vi "I2C Message Buffer - Check.vi"(8 "error in (no error)":errorcluster) -> (0 "error out":errorcluster, 2 "Messages":i32, 3 "Transactions":i32)   [LabVIEW 2025, in "I2C Bus Monitor.lvclass"]
uses:
  I2C Bus Monitor.lvclass
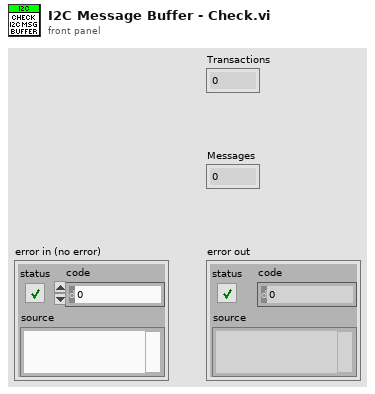
[diagram p1: front panel]
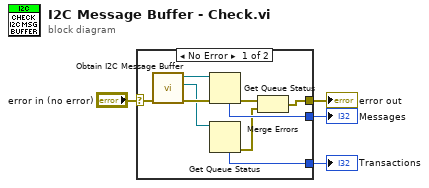
[diagram p0: block diagram]
diagram:
  n1 = case shown="No Error" "error in (no error)" {
    selector: "error in (no error)" -> [w8 w14]
    tunnel: [w13 _] -> w4
    tunnel: [w12 _] -> w3
    tunnel: [w10 w14] -> w2
    frame No Error {
      n2 = call "Obtain I2C Message Buffer.vi"("error in (no error)"=w8) -> ("error out"=w9:errorcluster, "Msgs per Txn Queue"=w7:refnum<queue>, "I2C Message Queue"=w6:refnum<queue>)  [unwired: 8 in]
      n3 = Get Queue Status(queue=w6, error in (no error)=w9) -> (error out=w11:errorcluster, # elements in queue=w13:i32)  [unwired: 1 in, 6 out]
      n4 = Get Queue Status(queue=w7) -> (error out=w5:errorcluster, # elements in queue=w12:i32)  [unwired: 2 in, 6 out]
      n5 = Merge Errors(w11, w5) -> (w10:errorcluster)
    }
    frame Error {
    }
  }
  "error out" <- w2
  "Messages" <- w4
  "Transactions" <- w3
